vi "Surveillance alarmes 1 2 3 4 reg.vi"() -> ()   [LabVIEW 2022 SP3]
uses:
  Enum/Enum r8.ctl
  Enum/Commande Choix arret reg.ctl
  Enum/Enum s1.ctl
  Variables globales/Variables glob EUROTHERM.vi
  Variables globales/Variable glob mails.vi
  Variables globales/Variable glob generale.vi
panel:
  out "Modif en cours":bool
  out "message mail":string
  out "Noms reg pb":string[](array[string])
  out "Dépassement seuil":T1(array[cluster])
  out "sortie d'erreur":errorcluster
  out "message":string
  out "AL OK nouveau":cluster{"AL OK 1 COM":u16[]}[](array[cluster]) {"AL OK 1 COM" items=["data = AL", "data pas nombre", "data diff. AL"]}
  out "problème":string
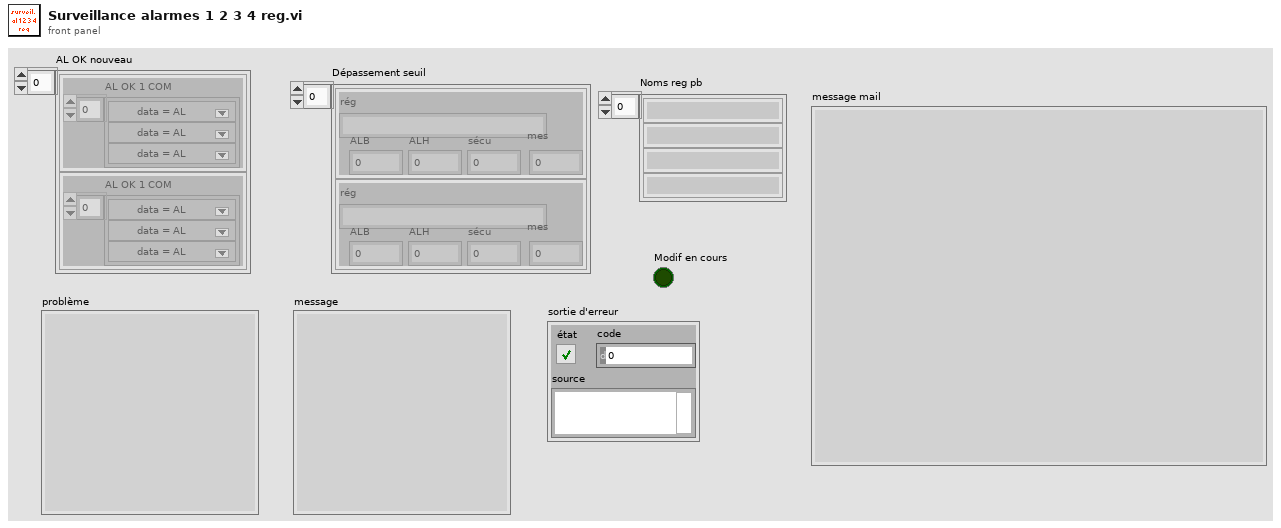
[diagram p1: front panel]
types:
  T1 = cluster{"rég":string, "mes":dbl, "ALB":dbl, "ALH":dbl, "sécu":dbl}[]
  T2 = typedef "Enum r8.ctl" = enum16{"init", "tempo", "lecture data", "AL enregistré a changé", "nouvelle alarme ?", "message hors gamme", "fin pb AL", "envoi AL et STOP", "message alerte AL", "mail alerte AL"}
  T3 = typedef "Enum s1.ctl" = enum16{"Alerte vide", "Alerte temperature min-max", "Alerte temperature ecart", "Alerte Keller", "Alerte compteur", "Alerte régulateurs"}
  T4 = cluster{"Noms voies select acqui 1COM":string[]}[]
  T5 = typedef "Commande Choix arret reg.ctl" = u16
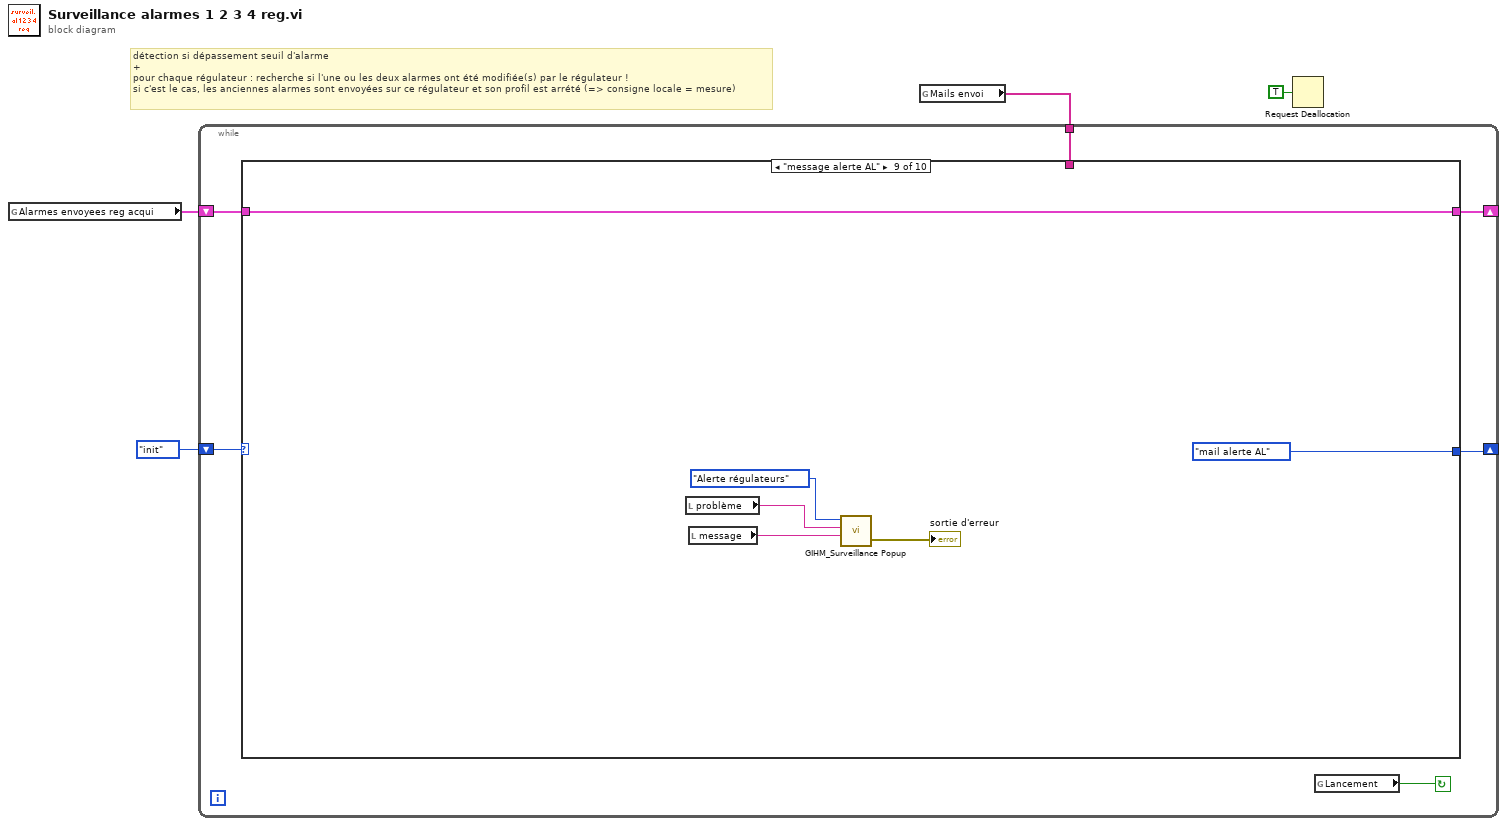
[diagram p0: block diagram]
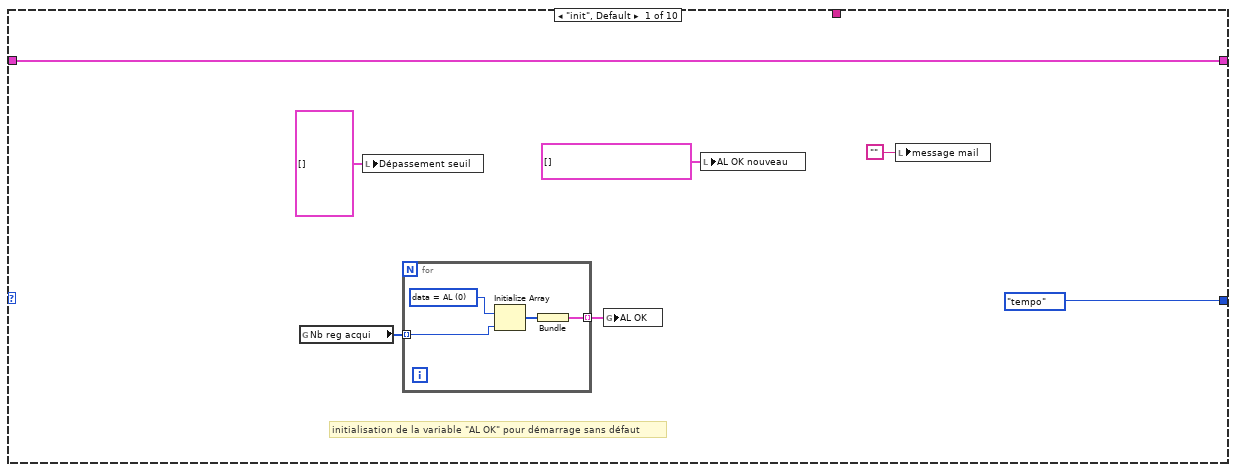
[diagram p2: hidden frame]
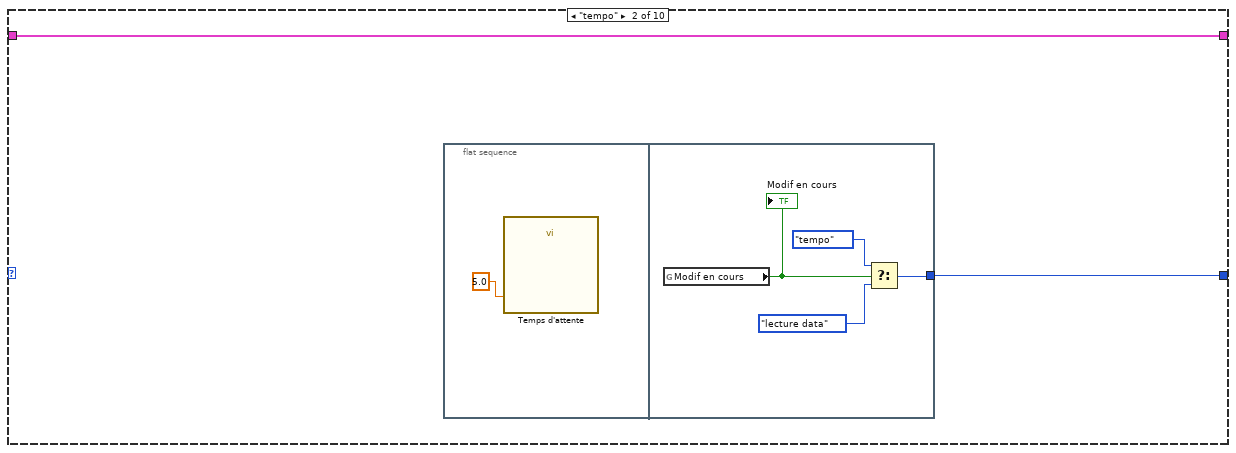
[diagram p3: hidden frame]
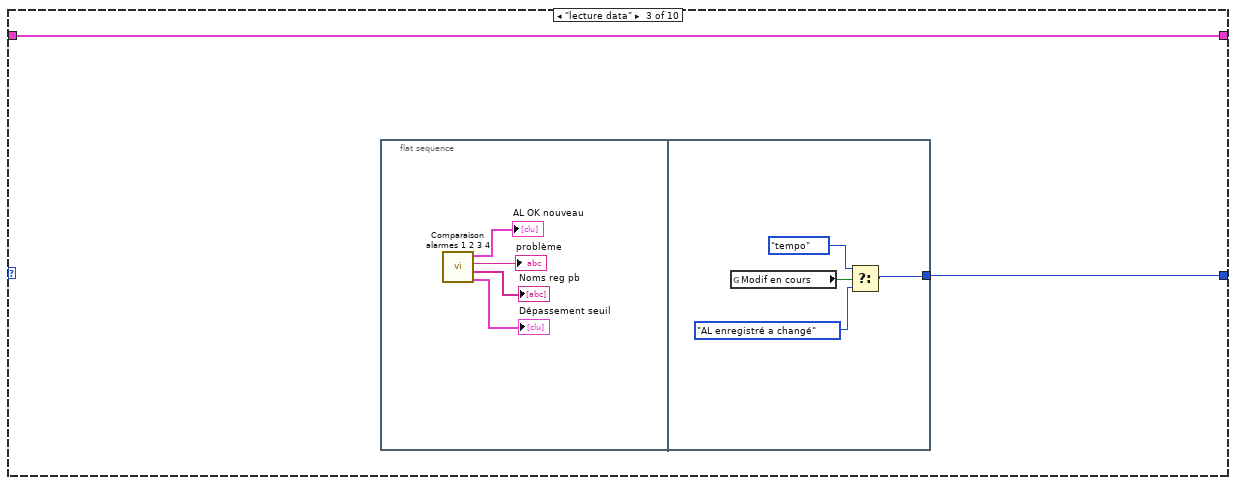
[diagram p4: hidden frame]
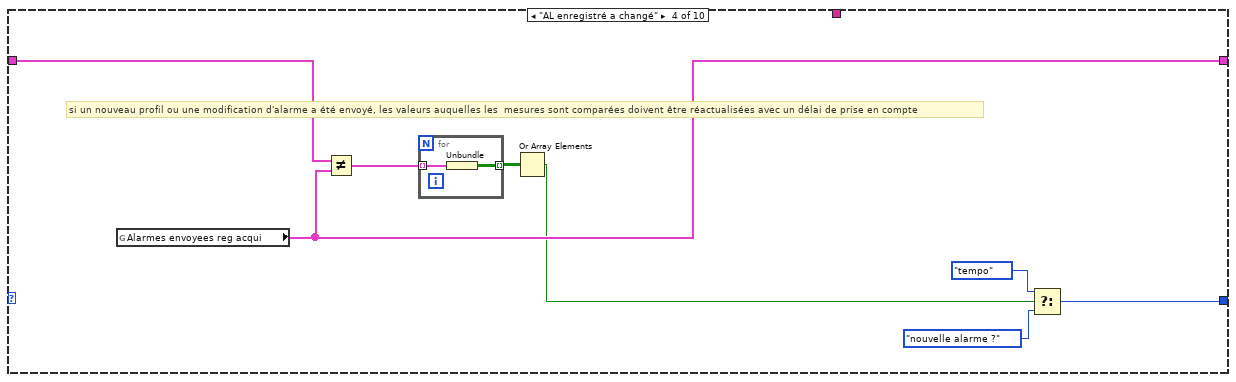
[diagram p5: hidden frame]
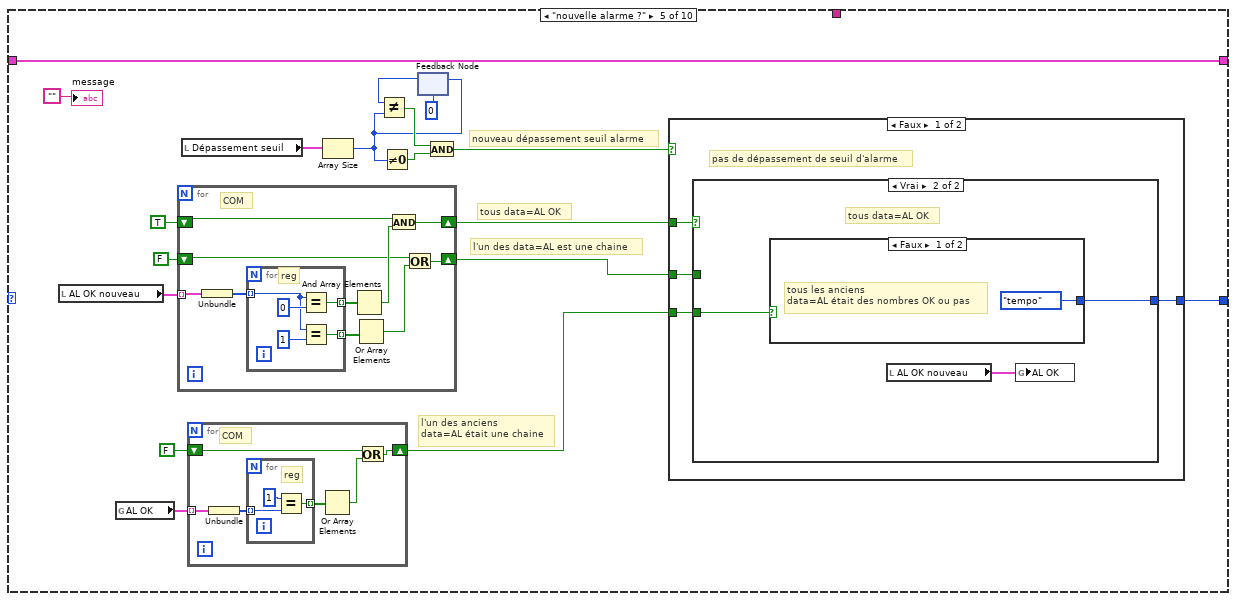
[diagram p6: hidden frame]
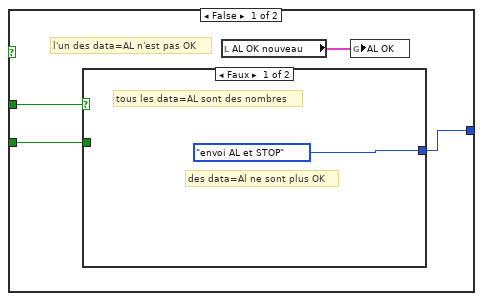
[diagram p7: hidden frame]
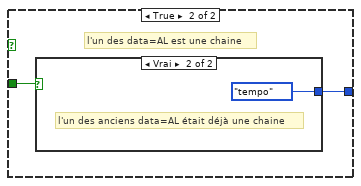
[diagram p8: hidden frame]
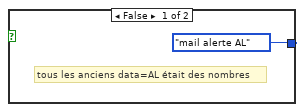
[diagram p9: hidden frame]
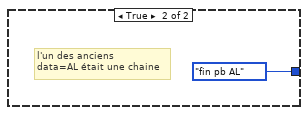
[diagram p10: hidden frame]
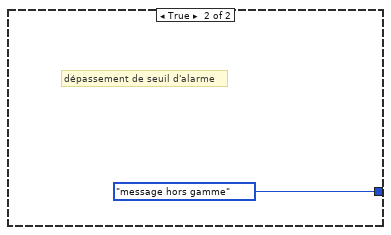
[diagram p11: hidden frame]
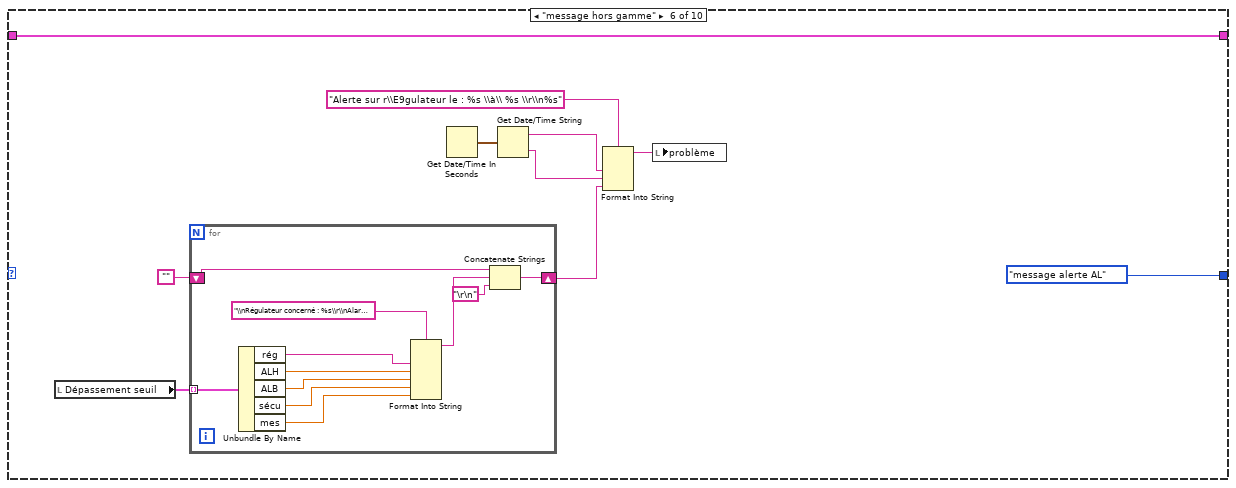
[diagram p12: hidden frame]
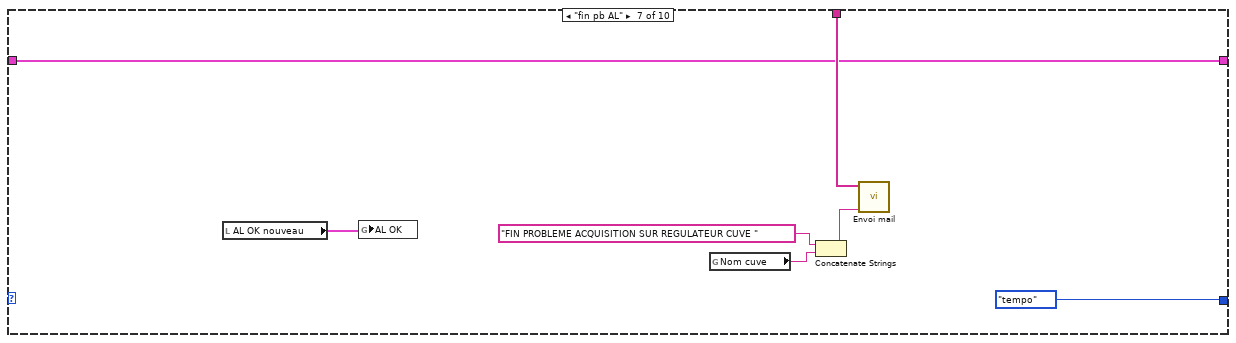
[diagram p13: hidden frame]
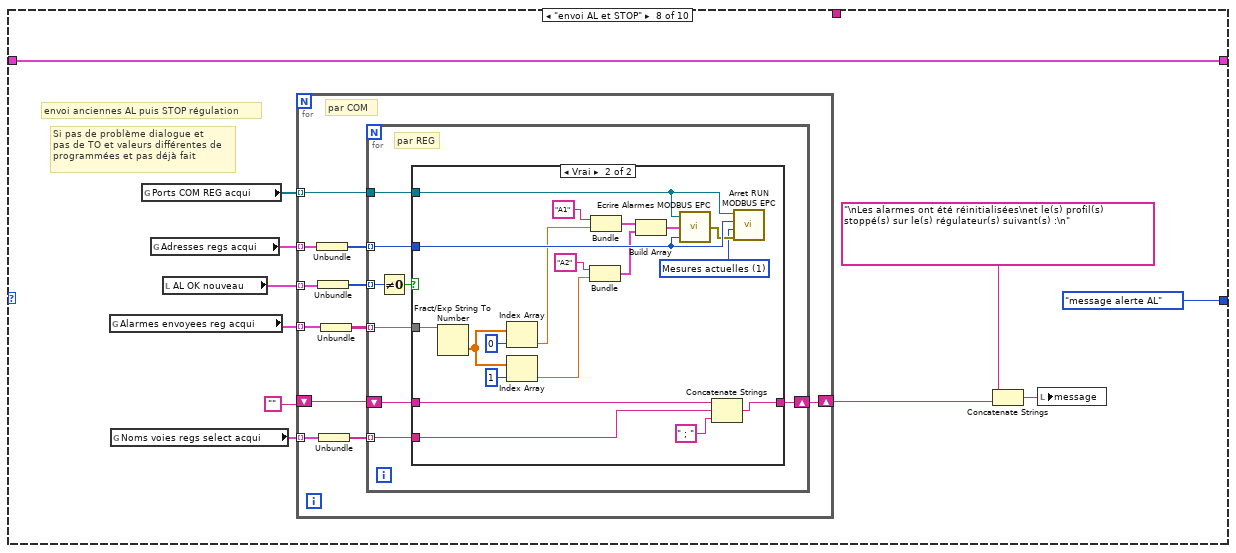
[diagram p14: hidden frame]
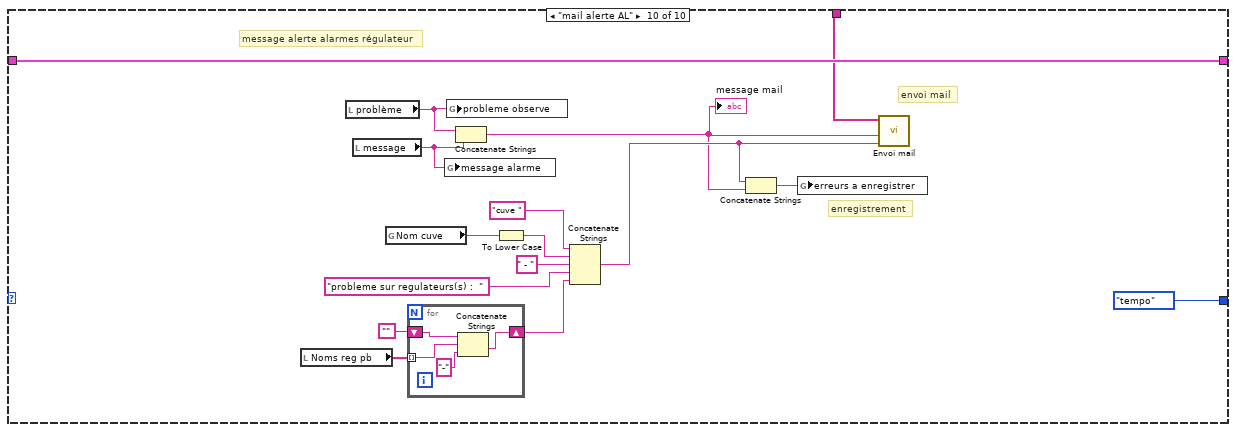
[diagram p16: hidden frame]
diagram:
  # "détection si dépassement seuil d'alarme\n+\npour chaque régulateur : recherche si l'une ou les deux alarmes ont été modifiée(s) par le régulateur !\nsi c'est le cas, les anciennes alarmes sont envoyées sur ce régulateur et son profil est arrété (=> consigne locale = mesure)"
  n1 = global read "Variables glob EUROTHERM.vi" "Alarmes envoyees reg acqui"() -> (w2:cluster{"alarmes 1COM reg":string[][]}[])
  n2 = global read "Variable glob mails.vi" "Mails envoi"() -> (w1:string[])
  n3 = while {
    shift-right: [w9] -> _
    shift-left: Enum_r8."init" ("Énum") -> [w10]
    tunnel: w1 -> [w7]
    shift-right: [w5] -> _
    shift-left: w2 -> [w6]
    stop <- w8 continue-if-true
    n4 = case shown="\"message alerte AL\"" w10 {
      tunnel: [Enum_r8."tempo" ("Énum") w22 w29 w39 w50 Enum_r8."message alerte AL" ("Énum") Enum_r8."tempo" ("Énum") Enum_r8."message alerte AL" ("Énum") Enum_r8."mail alerte AL" ("Énum") Enum_r8."tempo" ("Énum")] -> w9
      tunnel: w7 -> [_ _ _ _ _ _ w136 _ _ w197]
      tunnel: w6 -> [w14 w23 w30 w46 w62 w118 w131 w144 w191 w205]
      tunnel: [w14 w23 w30 w45 w62 w118 w131 w144 w191 w205] -> w5
      frame "init", Default {
        # "initialisation de la variable \"AL OK\" pour démarrage sans défaut"
        n5 = global read "Variables glob EUROTHERM.vi" "Nb reg acqui"() -> (w16:u8[])
        n6 = local write "Dépassement seuil"(T1 [] ("Dépassement seuil")) -> ()
        n7 = for {
          tunnel: w16 -> [w20] mode=indexing
          tunnel: [w18] -> w15 mode=indexing
          w21 = u16 0 items=["data = AL", "data pas nombre", "data diff. AL"] ("état AL")
          n8 = Initialize Array(w21, w20) -> (w19:u16[])
          n9 = Bundle(w19) -> (w18:cluster{u16[]})  [unwired: 1 in]
        }
        n10 = global write "Variables glob EUROTHERM.vi" "AL OK"(w15) -> ()
        n11 = local write "AL OK nouveau"(cluster{"AL OK 1 COM":u16[]}[] [] ("AL OK nouveau")) -> ()
        n12 = local write "message mail"("") -> ()
      }
      frame "tempo" {
        n13 = flat-sequence {
          tunnel: [w25] -> w22
          frame #0 {
            n14 = call "Temps d'attente"("Delay Time (s)"=5.0) -> ()  [unwired: 10 in, 1 out]
          }
          frame #1 {
            n15 = global read "Variables glob EUROTHERM.vi" "Modif en cours"() -> (w26:bool)
            "Modif en cours" <- w26
            n16 = Select(t=Enum_r8."tempo" ("Énum"), s=w26, f=Enum_r8."lecture data" ("Énum")) -> (s? t:f=w25:T2)
          }
        }
      }
      frame "lecture data" {
        n17 = flat-sequence {
          tunnel: [w35] -> w29
          frame #0 {
            n18 = call "Comparaison alarmes 1 2 3 4.vi"() -> ("AL OK nouveau"=→"AL OK nouveau":cluster{"AL OK 1 COM":u16[]}[], "problème"=→"problème":string, "regs pb"=→"Noms reg pb":string[], "Dépassement seuil"=→"Dépassement seuil":T1)  [unwired: 2 in]
          }
          frame #1 {
            n19 = global read "Variables glob EUROTHERM.vi" "Modif en cours"() -> (w36:bool)
            n20 = Select(t=Enum_r8."tempo" ("Énum"), s=w36, f=Enum_r8."AL enregistré a changé" ("Énum")) -> (s? t:f=w35:T2)
          }
        }
      }
      frame "AL enregistré a changé" {
        # "si un nouveau profil ou une modification d'alarme a été envoyé, les valeurs auquelles les  mesures sont comparées doivent être réactualisées avec un délai de prise en compte"
        n21 = global read "Variables glob EUROTHERM.vi" "Alarmes envoyees reg acqui"() -> (w45:cluster{"alarmes 1COM reg":string[][]}[])
        n22 = Not Equal?(x=w46, y=w45) -> (x != y?=w44:cluster{"alarmes 1COM reg":bool[][]}[])
        n23 = for {
          tunnel: w44 -> [w48] mode=indexing
          tunnel: [w47] -> w43 mode=indexing
          n24 = Unbundle(w48) -> ("alarmes 1COM reg"=w47:bool[][])
        }
        n25 = Or Array Elements(Boolean array=w43) -> (logical OR=w42:bool)
        n26 = Select(t=Enum_r8."tempo" ("Énum"), s=w42, f=Enum_r8."nouvelle alarme ?" ("Énum")) -> (s? t:f=w39:T2)
      }
      frame "nouvelle alarme ?" {
        # "nouveau dépassement seuil alarme"
        # "l'un des data=AL est une chaine"
        # "l'un des anciens \ndata=AL était une chaine"
        # "tous data=AL OK"
        n27 = local read "AL OK nouveau"() -> (w58:cluster{"AL OK 1 COM":u16[]}[])
        n28 = global read "Variables glob EUROTHERM.vi" "AL OK"() -> (w65:cluster{"AL OK 1 COM":u16[]}[])
        n29 = for {
          tunnel: w58 -> [w104] mode=indexing
          shift-right: [w98] -> w54
          shift-left: TRUE -> [w100]
          shift-right: [w95] -> w49
          shift-left: FALSE -> [w97]
          # "COM"
          n30 = Unbundle(w104) -> ("AL OK 1 COM"=w103:u16[])
          n31 = for {
            tunnel: w103 -> [w106] mode=indexing
            tunnel: [w108] -> w102 mode=indexing
            tunnel: [w105] -> w99 mode=indexing
            # "reg"
            n32 = Equal?(x=w106, y=u16 0) -> (x = y?=w108:bool)
            n33 = Equal?(x=w106, y=u16 1) -> (x = y?=w105:bool)
          }
          n34 = And Array Elements(Boolean array=w102) -> (logical AND=w101:bool)
          n35 = Or Array Elements(Boolean array=w99) -> (logical OR=w96:bool)
          n36 = And(x=w100, y=w101) -> (x .and. y?=w98:bool)
          n37 = Or(x=w97, y=w96) -> (x .or. y?=w95:bool)
        }
        n38 = local read "Dépassement seuil"() -> (w59:T1)
        n39 = for {
          tunnel: w65 -> [w91] mode=indexing
          shift-right: [w86] -> w53
          shift-left: FALSE -> [w87]
          # "COM"
          n40 = Unbundle(w91) -> ("AL OK 1 COM"=w90:u16[])
          n41 = for {
            tunnel: w90 -> [w94] mode=indexing
            tunnel: [w92] -> w89 mode=indexing
            # "reg"
            n42 = Equal?(x=u16 1, y=w94) -> (x = y?=w92:bool)
          }
          n43 = Or Array Elements(Boolean array=w89) -> (logical OR=w88:bool)
          n44 = Or(x=w87, y=w88) -> (x .or. y?=w86:bool)
        }
        n45 = Array Size(array=w59) -> (size(s)=w57:i32)
        n46 = Not Equal To 0?(x=w57) -> (x != 0?=w61:bool)
        n47 = feedback-in #1(w57) -> ()
        n48 = feedback #1(0) -> (w56:i32)
        n49 = Not Equal?(x=w56, y=w57) -> (x != y?=w60:bool)
        n50 = And(x=w60, y=w61) -> (x .and. y?=w51:bool)
        n51 = case shown="Faux" w51 {
          tunnel: w54 -> [w70 _]
          tunnel: w53 -> [w69 _]
          tunnel: [w68 Enum_r8."message hors gamme" ("Énum")] -> w50
          tunnel: w49 -> [w67 _]
          frame False {
            # "pas de dépassement de seuil d'alarme"
            n52 = case shown="Vrai" w70 {
              tunnel: [w74 w81] -> w68
              tunnel: w69 -> [w72 w80]
              tunnel: w67 -> [w71 _]
              frame False {
                # "l'un des data=AL n'est pas OK"
                n53 = case shown="Faux" w71 {
                  tunnel: [Enum_r8."envoi AL et STOP" ("Énum") w77] -> w74
                  tunnel: w72 -> [_ w76]
                  frame False {
                    # "des data=Al ne sont plus OK"
                    # "tous les data=AL sont des nombres"
                  }
                  frame True {
                    # "l'un des data=AL est une chaine"
                    n54 = case shown="Vrai" w76 {
                      tunnel: [Enum_r8."mail alerte AL" ("Énum") Enum_r8."tempo" ("Énum")] -> w77
                      frame False {
                        # "tous les anciens data=AL était des nombres"
                      }
                      frame True {
                        # "l'un des anciens data=AL était déjà une chaine"
                      }
                    }
                  }
                }
                n55 = local read "AL OK nouveau"() -> (w73:cluster{"AL OK 1 COM":u16[]}[])
                n56 = global write "Variables glob EUROTHERM.vi" "AL OK"(w73) -> ()
              }
              frame True {
                # "tous data=AL OK"
                n57 = case shown="Faux" w80 {
                  tunnel: [Enum_r8."tempo" ("Énum") Enum_r8."fin pb AL" ("Énum")] -> w81
                  frame False {
                    # "tous les anciens \ndata=AL était des nombres OK ou pas"
                  }
                  frame True {
                    # "l'un des anciens \ndata=AL était une chaine"
                  }
                }
                n58 = local read "AL OK nouveau"() -> (w82:cluster{"AL OK 1 COM":u16[]}[])
                n59 = global write "Variables glob EUROTHERM.vi" "AL OK"(w82) -> ()
              }
            }
          }
          frame True {
            # "dépassement de seuil d'alarme"
          }
        }
        "message" <- ""
      }
      frame "message hors gamme" {
        n60 = local read "Dépassement seuil"() -> (w117:T1)
        n61 = for {
          tunnel: w117 -> [w130] mode=indexing
          shift-right: [w123] -> w110
          shift-left: "" -> [w122]
          n62 = Unbundle By Name(w130) -> ("rég"=w125:string, "ALH"=w126:dbl, "ALB"=w129:dbl, "sécu"=w128:dbl, "mes"=w127:dbl)
          n63 = Format Into String(format string="\\nRégulateur concerné : %s\\r\\nAlarme haute : %.2f\\rAlarme basse : %.2f\\r\\nLes valeurs mesurée sont  :\\rPt \"sécurité\" = %.2f\\rPt \"mesure\" = %.2f\\r\\n" ("chaîne de format"), w125, w126, w129, w128, w127) -> (resulting string=w121:string)  [unwired: 2 in, 1 out]
          n64 = Concatenate Strings(w122, w121, "\r\n") -> (w123:string)
        }
        n65 = Get Date/Time In Seconds() -> (seconds since 1Jan1904=w116:timestamp)
        n66 = Get Date/Time String(seconds (now)=w116) -> (date string=w115:string, time string=w114:string)  [unwired: 2 in]
        n67 = Format Into String(format string="Alerte sur r\\E9gulateur le : %s \\à\\ %s \\r\\n%s", w115, w114, w110) -> (resulting string=w112:string)  [unwired: 2 in, 1 out]
        n68 = local write "problème"(w112) -> ()
      }
      frame "fin pb AL" {
        n69 = local read "AL OK nouveau"() -> (w132:cluster{"AL OK 1 COM":u16[]}[])
        n70 = global write "Variables glob EUROTHERM.vi" "AL OK"(w132) -> ()
        n71 = global read "Variable glob generale.vi" "Nom cuve"() -> (w134:string)
        n72 = Concatenate Strings("FIN PROBLEME ACQUISITION SUR REGULATEUR CUVE ", w134) -> (w133:string)
        n73 = call "Envoi mail.vi"("Objet"=w133, "Mail liste"=w136) -> ()  [unwired: 4 in]
      }
      frame "envoi AL et STOP" {
        # "Si pas de problème dialogue et\npas de TO et valeurs différentes de\nprogrammées et pas déjà fait"
        # "envoi anciennes AL puis STOP régulation"
        n74 = global read "Variables glob EUROTHERM.vi" "Alarmes envoyees reg acqui"() -> (w145:cluster{"alarmes 1COM reg":string[][]}[])
        n75 = global read "Variables glob EUROTHERM.vi" "Noms voies regs select acqui"() -> (w142:T4)
        n76 = global read "Variables glob EUROTHERM.vi" "Ports COM REG acqui"() -> (w147:refnum<visa-resource-name>[])
        n77 = global read "Variables glob EUROTHERM.vi" "Adresses regs acqui"() -> (w146:cluster{"Adresses acqui 1COM reg":u16[]}[])
        n78 = local read "AL OK nouveau"() -> (w138:cluster{"AL OK 1 COM":u16[]}[])
        n79 = for {
          tunnel: w147 -> [w159] mode=indexing
          tunnel: w146 -> [w158] mode=indexing
          tunnel: w145 -> [w156] mode=indexing
          tunnel: w142 -> [w154] mode=indexing
          shift-right: [w151] -> w139
          shift-left: "" -> [w152]
          tunnel: w138 -> [w150] mode=indexing
          # "par COM"
          n80 = Unbundle(w158) -> ("Adresses acqui 1COM reg"=w157:u16[])
          n81 = Unbundle(w150) -> ("AL OK 1 COM"=w149:u16[])
          n82 = Unbundle(w154) -> ("Noms voies select acqui 1COM"=w153:string[])
          n83 = Unbundle(w156) -> ("alarmes 1COM reg"=w155:string[][])
          n84 = for {
            tunnel: w159 -> [w167]
            tunnel: w157 -> [w166] mode=indexing
            tunnel: w155 -> [w165] mode=indexing
            tunnel: w153 -> [w163] mode=indexing
            shift-right: [w162] -> w151
            shift-left: w152 -> [w164]
            tunnel: w149 -> [w161] mode=indexing
            # "par REG"
            n85 = Not Equal To 0?(x=w161) -> (x != 0?=w160:bool)
            n86 = case shown="Vrai" w160 {
              tunnel: w167 -> [_ w187]
              tunnel: w166 -> [_ w186]
              tunnel: w165 -> [_ w185]
              tunnel: w164 -> [w168 w173]
              tunnel: w163 -> [_ w172]
              tunnel: [w168 w170] -> w162
              frame False {
              }
              frame True {
                w169 = T5 1 items=["Consignes actuelles", "Mesures actuelles", "Valeur fixe pour tous les régulateurs"] ("Choix consigne locale :")
                n87 = Fract/Exp String To Number(string=w185) -> (number=w178:dbl[])  [unwired: 3 in, 1 out]
                n88 = Index Array(array=w178, index=0 ("indice")) -> (element=w175:dbl)
                n89 = Index Array(array=w178, index=1 ("indice")) -> (element=w174:dbl)
                n90 = Bundle("A2", "Chaîne"=w174) -> (w182:cluster{string, "Chaîne":dbl})  [unwired: 1 in]
                n91 = Bundle("A1", "Chaîne"=w175) -> (w181:cluster{string, "Chaîne":dbl})  [unwired: 1 in]
                n92 = Build Array(w181, w182) -> (w183:cluster{string, "Chaîne":dbl}[])
                n93 = call "Ecrire Alarmes MODBUS EPC.vi"("Adresse rég"=w186, "Programmation configuration"=w183, "Port COM run 1 REG"=w187) -> ("error out"=w184:errorcluster)
                n94 = Concatenate Strings(w173, w172, " ; ") -> (w170:string)
                n95 = call "Arret RUN MODBUS EPC.vi"("Port COM run 1 REG"=w187, "Adresse"=w186, "Choix consigne locale :"=w169, "error in"=w184) -> ()  [unwired: 2 in, 2 out]
              }
            }
          }
        }
        n96 = Concatenate Strings("\nLes alarmes ont été réinitialisées\net le(s) profil(s) stoppé(s) sur le(s) régulateur(s) suivant(s) :\n", w139) -> (w143:string)
        n97 = local write "message"(w143) -> ()
      }
      frame "message alerte AL" {
        n98 = local read "problème"() -> (w190:string)
        n99 = local read "message"() -> (w189:string)
        n100 = call "GIHM_Surveillance Popup.vi"("Message"=w189, "Problème observé"=w190, "Type problème"=Enum_s1."Alerte régulateurs") -> ("error out"=→"sortie d'erreur":errorcluster)  [unwired: 2 in]
      }
      frame "mail alerte AL" {
        # "enregistrement"
        # "envoi mail"
        # "message alerte alarmes régulateur"
        n101 = local read "Noms reg pb"() -> (w202:string[])
        n102 = local read "problème"() -> (w206:string)
        n103 = local read "message"() -> (w207:string)
        n104 = global read "Variable glob generale.vi" "Nom cuve"() -> (w199:string)
        n105 = for {
          tunnel: w202 -> [w213] mode=indexing
          shift-right: [w212] -> w200
          shift-left: "" -> [w211]
          n106 = Concatenate Strings(w211, w213, "-" ("chaîne")) -> (w212:string)
        }
        n107 = global write "Variables glob EUROTHERM.vi" "message alarme"(w207) -> ()
        n108 = global write "Variables glob EUROTHERM.vi" "probleme observe"(w206) -> ()
        n109 = Concatenate Strings(w206, w207) -> (w195:string)
        "message mail" <- w195
        n110 = To Lower Case(string=w199) -> (all lower case string=w198:string)
        n111 = Concatenate Strings("cuve ", w198, " - " ("chaîne"), "probleme sur regulateurs(s) :  ", w200) -> (w196:string)
        n112 = Concatenate Strings(w196, w195) -> (w194:string)
        n113 = global write "Variable glob generale.vi" "erreurs a enregistrer"(w194) -> ()
        n114 = call "Envoi mail.vi"("Objet"=w196, "Message"=w195, "Mail liste"=w197) -> ()  [unwired: 3 in]
      }
    }
    n115 = global read "Variable glob generale.vi" "Lancement"() -> (w8:bool)
  }
  n116 = Request Deallocation(TRUE ("flag")) -> ()
